vi "AIT 429 - Add Data Channel.vi"(8 "error in (no error)":errorcluster, 11 "Node Ptr":u64 format="%.0x") -> (0 "error out":errorcluster)   [LabVIEW 2015, in "AIT 429 System Explorer.lvlib"]
uses:
  <vilib>/NI Veristand/Custom Device API/Custom Device Channel.ctl
  <vilib>/NI Veristand/Custom Device API/Custom Device Channel Type.ctl
  Shared/Controls and Global/Global.vi
  <vilib>/NI Veristand/Custom Device API/Get Item Property (U32).vi
  AIT 429 System Explorer.lvlib
  Shared/AIT 429 Shared.lvlib
  <vilib>/NI Veristand/Custom Device API/Custom Device API.lvlib
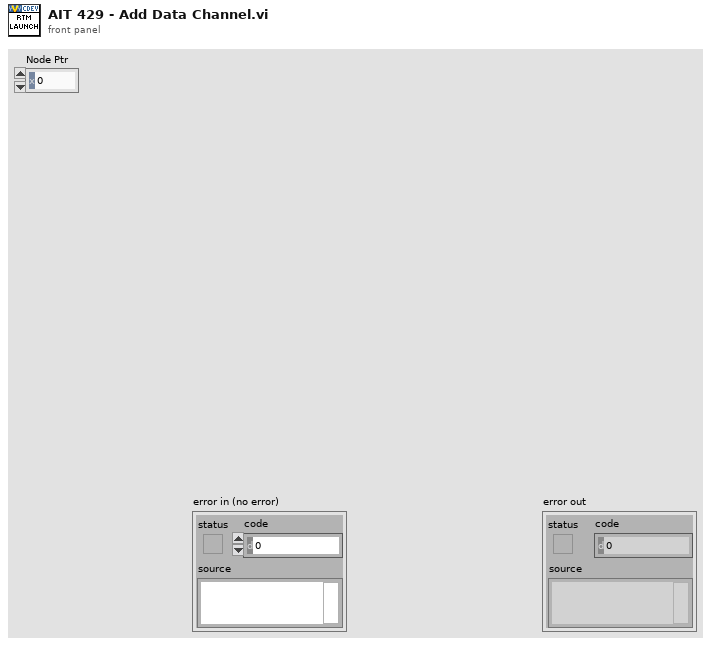
[diagram p1: front panel]
types:
  T1 = typedef "Custom Device API.lvlib/Custom Device Channel Type.ctl" = enum16{"Input", "Output"}
  T2 = typedef "Custom Device API.lvlib/Custom Device Channel.ctl" = cluster{"Type":T1, "Units":string, "Default Value":dbl, "Faultable":bool, "Scalable":bool}
  T3 = typedef "Custom Device API.lvlib/Custom Device Item Ref.ctl" = u64
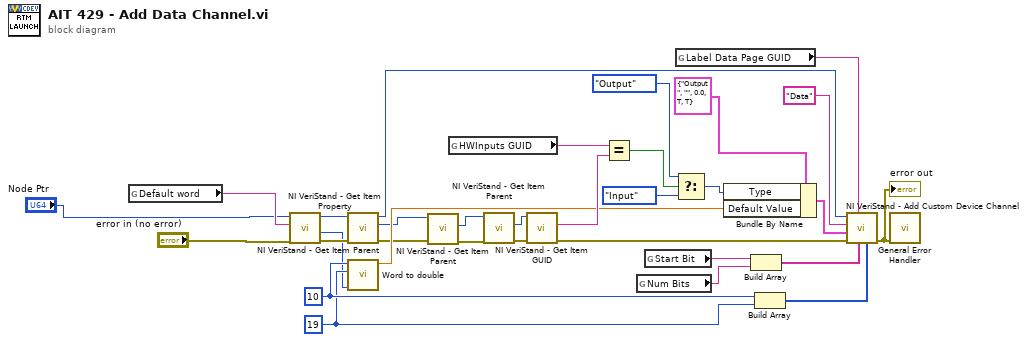
[diagram p0: block diagram]
diagram:
  w11 = 19
  w12 = 10
  n1 = global read "Global.vi" "Default word"() -> (w8:string)
  n2 = call-poly <vilib>:"NI VeriStand - Get Item Property.vi"("error in (no error)"="error in (no error)", "Property Name"=w8, "Item Ref in"="Node Ptr") -> ("error out"=w9:errorcluster, "Value"=w7:u32, "Item Ref out"=w10:T3)  [unwired: 5 in, 1 out]
  n3 = call <vilib>:"NI VeriStand - Get Item Parent.vi"("error in (no error)"=w9, "Item Ref in"=w10) -> ("error out"=w2:errorcluster, "Parent Ref"=w4:T3, "Item Ref out"=w22:T3)  [unwired: 6 in, 1 out]
  n4 = call "Word to double.vi"("word"=w7, "Number of Bits"=w11, "Start Bit"=w12) -> ("Double"=w13:dbl)  [unwired: 8 in]
  n5 = call <vilib>:"NI VeriStand - Get Item Parent.vi"("error in (no error)"=w2, "Item Ref in"=w4) -> ("error out"=w1:errorcluster, "Parent Ref"=w3:T3)  [unwired: 6 in, 2 out]
  n6 = global read "Global.vi" "HWInputs GUID"() -> (w24:string)
  n7 = call <vilib>:"NI VeriStand - Get Item Parent.vi"("error in (no error)"=w1, "Item Ref in"=w3) -> ("error out"=w30:errorcluster, "Parent Ref"=w29:T3)  [unwired: 6 in, 2 out]
  n8 = call <vilib>:"NI VeriStand - Get Item GUID.vi"("error in (no error)"=w30, "Item Ref in"=w29) -> ("error out"=w17:errorcluster, "GUID"=w23:string)  [unwired: 7 in, 1 out]
  n9 = Equal?(x=w24, y=w23) -> (x = y?=w19:bool)
  n10 = global read "Global.vi" "Num Bits"() -> (w32:string)
  n11 = global read "Global.vi" "Start Bit"() -> (w20:string)
  n12 = global read "Global.vi" "Label Data Page GUID"() -> (w31:string)
  n13 = Select(t=Custom_Device_Channel_Type."Output" ("Type"), s=w19, f=Custom_Device_Channel_Type."Input" ("Type")) -> (s? t:f=w27:T1)
  n14 = Bundle By Name(cluster=T2 {"Type"=enum."Output", "Units"="", "Default Value"=0.0, "Faultable"=TRUE, "Scalable"=TRUE} ("Channel"), "Type"=w27, "Default Value"=w13) -> (w15:T2)
  n15 = Build Array(w20, w32) -> (w21:string[])
  n16 = Build Array(w12, w11) -> (w16:i32[])
  n17 = call <vilib>:"NI VeriStand - Add Custom Device Channel.vi"("Property Values"=w16, "Property names"=w21, "GUID (Default Channel)"=w31, "error in (no error)"=w17, "Channel"=w15, "Channel Name"="Data", "Parent Ref in"=w22) -> ("error out"=w18:errorcluster)  [unwired: 1 in, 3 out]
  "error out" <- w18
  n18 = call <vilib>:"General Error Handler.vi"("error in (no error)"=w18) -> ()  [unwired: 10 in, 5 out]
